vi "Cascade Controller.vi"(8 "error in":errorcluster) -> ()   [LabVIEW 2027]
doc: "This VI responds to drive commands both auto and tele Opmodes.\nIt owns the drivebase motors and sensors and runs independent from opModes. Commands can run for arbitrary times, but newly posted commands will interupt as long as Check is called and used for time delays."
uses:
  <vilib>/Rock Robotics/WPI/Framework/Completion Status.ctl
  Cascade Setpoints.ctl
  Cascade Operations.ctl
  Cascade Positions.ctl
  <vilib>/REV Custom Controls/SPARK Closed Loop Slot.ctl
  <vilib>/REV Custom Controls/Spark Output Control Type.ctl
  <vilib>/MRC/Types/CmdCtl Completion.ctl
  <vilib>/REVLibDriver/REVLibDriver.lvlib
  <resource>/objmgr/REVSpark.rc
  bef5a86c-5ad3-3fec-b018-693a5248eb3f.vi
panel:
  in  "Closed Loop Slot":T1 items=["Slot 0", "Slot 1", "Slot 2", "Slot 3"]
  in  "PID Gains":T2
  in  "PID Gains 2 VEL":T2={{"P Gain"=0.0001, "I Gain"=0.0, "D Gain"=0.0, "kV"=0.002}, "I Zone"=0.0, "Output LImits"={"Min Output"=-0.7, "Max Output"=0.7}}
  in  "PID Gains POS":T2
  in  "Abort Cmd":bool
  in  "Execute Cmd":bool
  in  "Interactive Values":T3
  out "Command Timing":cluster{"Start Time (ms)":u32, "Iterations":i32}
  out "Status":T6
  out "Current Command Data":T3
  out "Cmd Summary":string
  # "Interactive Command: You may fill in the settings for a command\nand schedule it with the Execute button. You can observe and abort\nany command while fine tuning the code for the controller."
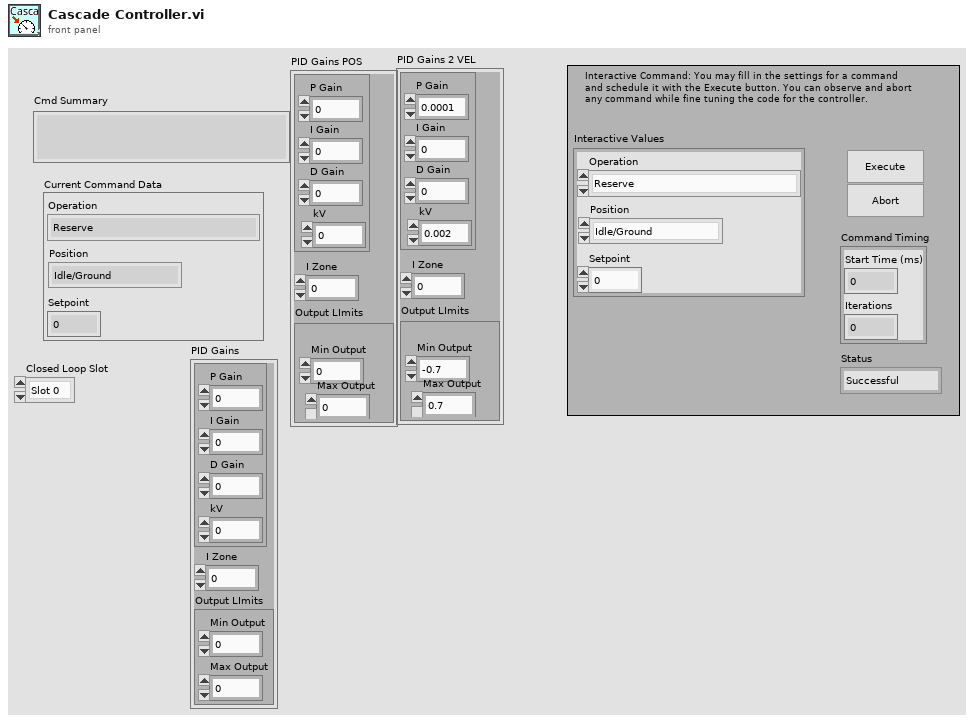
[diagram p1: front panel]
types:
  T1 = typedef "SPARK Closed Loop Slot.ctl" = u16
  T2 = cluster{cluster{"P Gain":dbl, "I Gain":dbl, "D Gain":dbl, "kV":dbl}, "I Zone":dbl, "Output LImits":cluster{"Min Output":dbl, "Max Output":dbl}}
  T3 = typedef "Cascade Setpoints.ctl" = cluster{"Operation":T4, "Position":T5, "Setpoint":dbl}
  T4 = typedef "Cascade Operations.ctl" = enum16{"Reserve", "Read Current", "Immediate", "State Machine"}
  T5 = typedef "Cascade Positions.ctl" = enum16{"Idle/Ground", "Raised L1", "L2", "L2 Tip", "L3", "L3 Tip", "Feeder", "\"Default\""}
  T6 = typedef "Completion Status.ctl" = enum16{"Successful", "Aborted", "Incomplete"}
  T7 = typedef "REVLibDriver.lvlib/REVSparkRefnum.ctl" = refnum<k20>
  T8 = typedef "Command Status Info.ctl" = cluster{"Name":string, "Status":T6, "notifier out":T9}
  T9 = typedef "Completion Notifier.ctl" = refnum<notifier>
  T10 = cluster{"Current Command":T3, "Command Timing":cluster{"Start Time (ms)":u32, "Iterations":i32}, "Command Arguments":cluster{"Command Info":T8, "Description":string, "Default Command":T3, "queue out":refnum<queue>, "Subsystem Name":string}}
  T11 = typedef "REVLibDriver.lvlib/Spark Output Control Type.ctl" = enum16{"Percent VBus", "Velocity", "Voltage", "Position", "Current", "MAXMotion Position", "MAXMotion Velocity"}
  T12 = typedef "CmdCtl Completion.ctl" = enum16{"incomplete", "finished"}
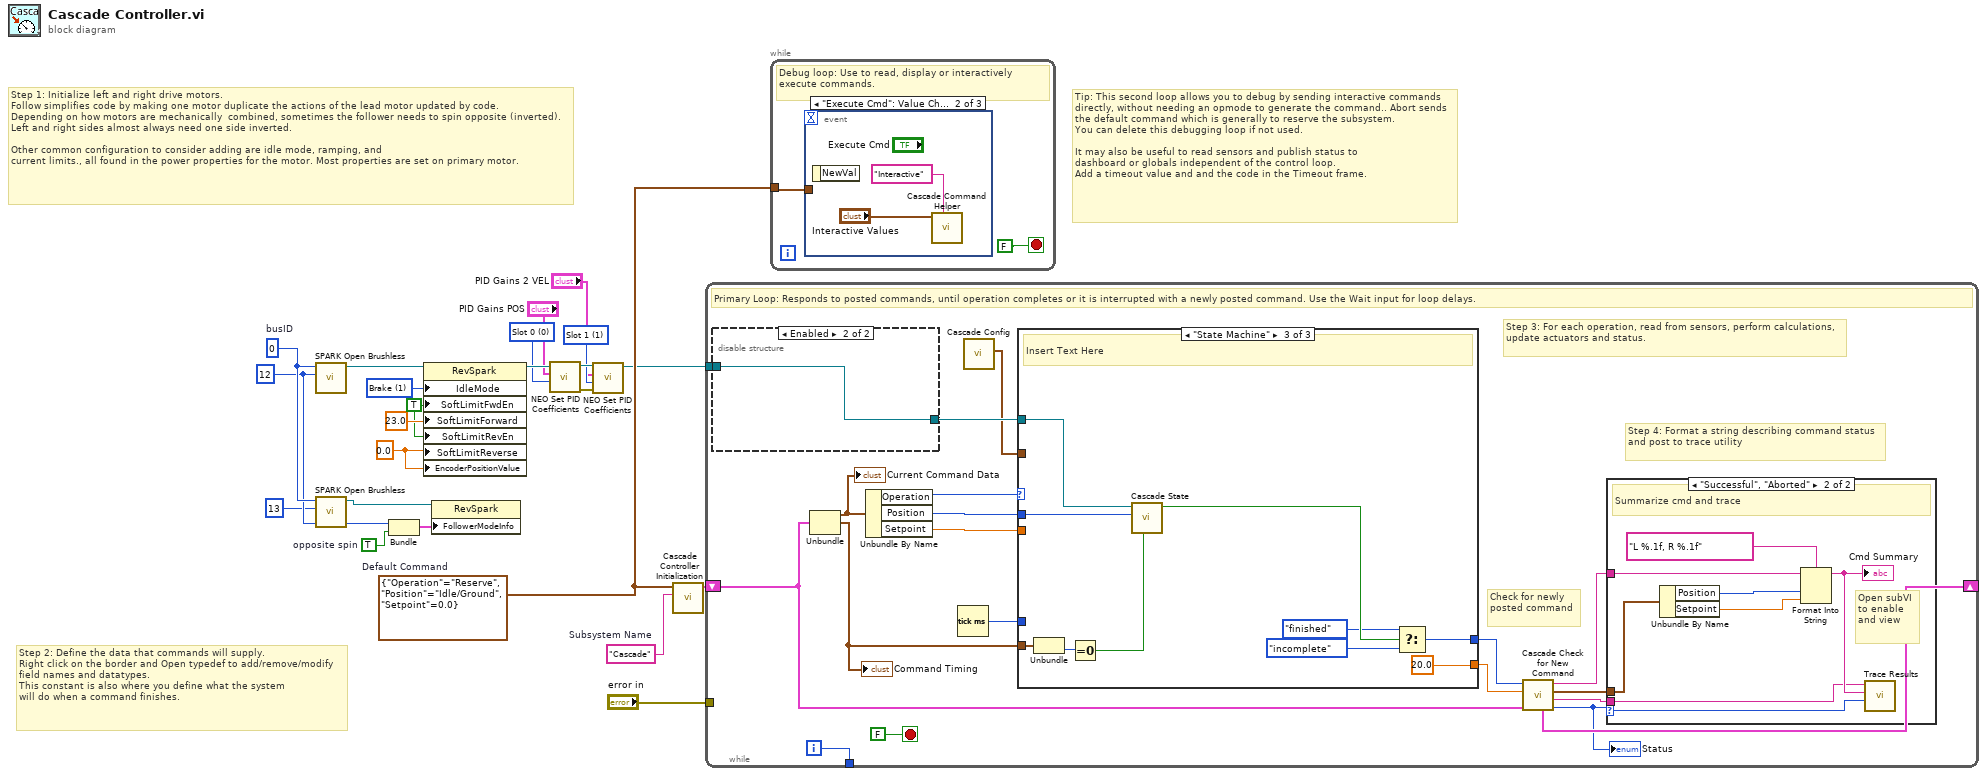
[diagram p0: block diagram]
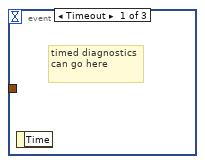
[diagram p2: hidden frame]
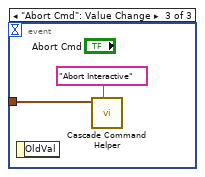
[diagram p3: hidden frame]
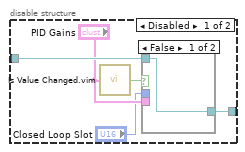
[diagram p4: hidden frame]
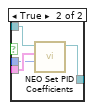
[diagram p5: hidden frame]
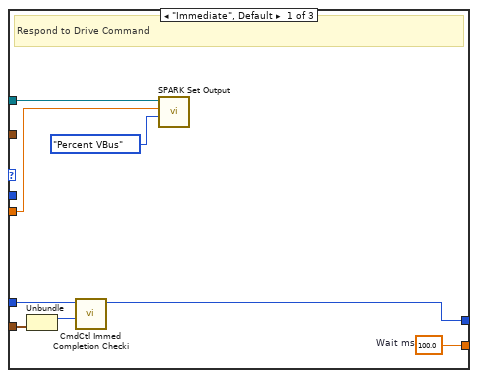
[diagram p7: hidden frame]
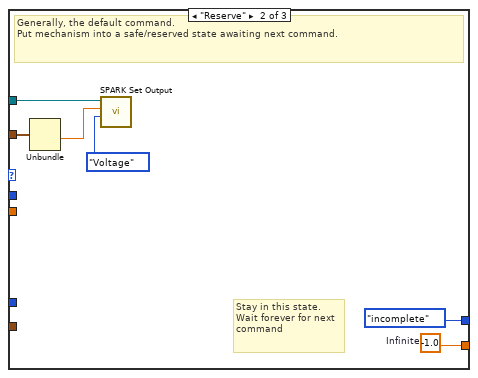
[diagram p8: hidden frame]
diagram:
  w5 = T1 1 items=["Slot 0", "Slot 1", "Slot 2", "Slot 3"] ("Closed Loop Slot")
  w2 = sgl 0.0 ("SoftLimitReverse")
  w1 = TRUE ("SoftLimitFwdEn")
  w10 = T1 0 items=["Slot 0", "Slot 1", "Slot 2", "Slot 3"] ("Closed Loop Slot")
  w12 = u32 1 items=["Coast", "Brake"] ("IdleMode")
  w17 = TRUE  # opposite spin
  w20 = 0  # busID
  w14 = 12
  w19 = T3 {"Operation"=enum."Reserve", "Position"=enum."Idle/Ground", "Setpoint"=0.0}  # Default Command
  w21 = "Cascade"  # Subsystem Name
  # "Tip: This second loop allows you to debug by sending interactive commands\ndirectly, without needing an opmode to generate the command.. Abort sends\nthe default command which is generally to reserve the subsystem.\nYou can delete this debugging loop if not used.\n\nIt may also be useful to read sensors and publish status to\ndashboard or globals independent of the control loop.\nAdd a timeout value and and the code in the Timeout frame."
  # "Step 2: Define the data that commands will supply.\nRight click on the border and Open typedef to add/remove/modify\nfield names and datatypes.\nThis constant is also where you define what the system\nwill do when a command finishes."
  # "Step 1: Initialize left and right drive motors.\nFollow simplifies code by making one motor duplicate the actions of the lead motor updated by code.\nDepending on how motors are mechanically  combined, sometimes the follower needs to spin opposite (inverted).\nLeft and right sides almost always need one side inverted.\n\nOther common configuration to consider adding are idle mode, ramping, and\ncurrent limits., all found in the power properties for the motor. Most properties are set on primary motor."
  n1 = call <vilib>:"SPARK Open Brushless.vi"("deviceId"=w14, "busID"=w20) -> ("Spark refnum"=w18:T7)  [unwired: 8 in, 1 out]
  n2 = call <vilib>:"SPARK Open Brushless.vi"("deviceId"=13, "busID"=w20) -> ("Spark refnum"=w16:T7)  [unwired: 8 in, 1 out]
  n3 = Bundle(w14, "opposite spin"=w17) -> (w15:cluster{i32, "opposite spin ":bool})  [unwired: 1 in]
  n4 = property class="RevSpark"(reference=w18, "IdleMode"=w12, "SoftLimitFwdEn"=w1, "SoftLimitForward"=sgl 23.0, "SoftLimitRevEn"=w1, "SoftLimitReverse"=w2, "EncoderPositionValue"=w2) -> (reference out=w11:T7)  [unwired: 1 in, 1 out]
  n5 = property class="RevSpark"(reference=w16, "FollowerModeInfo"=w15) -> ()  [unwired: 1 in, 2 out]
  n6 = call "NEO Set PID Coefficients.vi"("Closed Loop Slot"=w10, "PID Gains"="PID Gains POS", "Spark refnum"=w11) -> ("error out"=w7:errorcluster, "Spark refnum out"=w6:T7)  [unwired: 5 in]
  n7 = call "NEO Set PID Coefficients.vi"("error in"=w7, "Closed Loop Slot"=w5, "PID Gains"="PID Gains 2 VEL", "Spark refnum"=w6) -> ("Spark refnum out"=w3:T7)  [unwired: 4 in, 1 out]
  n8 = call "Cascade Controller Initialization.vi"("Subsystem Name"=w21, "Default Command"=w19) -> ("Current Command"=w22:T10)  [unwired: 9 in]
  n9 = while {
    shift-right: [w36] -> _
    shift-left: w22 -> [w30]
    tunnel: [w41] -> _
    tunnel: "error in" -> [_]
    tunnel: w3 -> [w26]
    i -> [w41]
    stop <- FALSE stop-if-true
    # "Step 4: Format a string describing command status\nand post to trace utility"
    # "Check for newly\nposted command"
    # "Step 3: For each operation, read from sensors, perform calculations,\nupdate actuators and status."
    # "Primary Loop: Responds to posted commands, until operation completes or it is interrupted with a newly posted command. Use the Wait input for loop delays."
    n10 = disable-structure shown="Enabled" {
      disable-tunnel: w26 -> [w47 w53]
      disable-tunnel: [w46 w53] -> w25
      frame Disabled {
        n11 = call "Is Value Changed.vim"("value"="PID Gains") -> ("changed or first call?"=w45:bool)
        n12 = case shown="False" w45 {
          tunnel: w47 -> [w48 w52]
          tunnel: [w48 w51] -> w46
          tunnel: "PID Gains" -> [_ w50]
          tunnel: "Closed Loop Slot" -> [_ w49]
          frame False {
          }
          frame True {
            n13 = call "NEO Set PID Coefficients.vi"("Closed Loop Slot"=w49, "PID Gains"=w50, "Spark refnum"=w52) -> ("Spark refnum out"=w51:T7)  [unwired: 5 in, 1 out]
          }
        }
      }
      frame Enabled {
      }
    }
    n14 = Unbundle(w30) -> ("Current Command"=w28:T3, "Command Timing"=w29:cluster{"Start Time (ms)":u32, "Iterations":i32})  [unwired: 1 out]
    "Command Timing" <- w29
    "Current Command Data" <- w28
    n15 = Unbundle By Name(w28) -> ("Operation"=w40:T4, "Position"=w39:T5, "Setpoint"=w37:dbl)
    n16 = Tick Count (ms)() -> (millisecond timer value=w38:u32)
    n17 = call "Cascade Config.vi"() -> ("FeedForward Constants Out"=w24:cluster{"kA":dbl, "kS":dbl, "kG":dbl, "kV":dbl})  [unwired: 10 in, 1 out]
    n18 = case shown="\"State Machine\"" w40 {
      tunnel: [w69 w75 20.0 ("Infinite")] -> w34
      tunnel: [w66 CmdCtl_Completion."incomplete" w81] -> w35
      tunnel: w29 -> [w68 _ w78]
      tunnel: w39 -> [_ _ w79]
      tunnel: w38 -> [w67 _ _]
      tunnel: w37 -> [w62 _ _]
      tunnel: w25 -> [w63 w73 w85]
      tunnel: w24 -> [_ w72 _]
      frame "Immediate", Default {
        w69 = 100.0  # Wait ms
        # "Respond to Drive Command"
        n19 = Unbundle(w68) -> ("Start Time (ms)"=w65:u32)  [unwired: 1 out]
        n20 = call <vilib>:"CmdCtl Immed Completion Checki.vi"("Start Time (ms)"=w65, "current time (ms)"=w67) -> ("Completion"=w66:T12)  [unwired: 9 in]
        n21 = call <vilib>:"SPARK Set Output.vi"("Control Mode"=Spark_Output_Control_Type."Percent VBus", "Setpoint"=w62, "Spark refnum"=w63) -> ()  [unwired: 7 in, 2 out]
      }
      frame "Reserve" {
        w75 = -1.0  # Infinite
        # "Stay in this state.\nWait forever for next\ncommand"
        # "Generally, the default command.\nPut mechanism into a safe/reserved state awaiting next command."
        n22 = Unbundle(w72) -> ("kG"=w71:dbl)  [unwired: 3 out]
        n23 = call <vilib>:"SPARK Set Output.vi"("Control Mode"=Spark_Output_Control_Type."Voltage", "Setpoint"=w71, "Spark refnum"=w73) -> ()  [unwired: 7 in, 2 out]
      }
      frame "State Machine" {
        # "Insert Text Here"
        n24 = Unbundle(w78) -> ("Iterations"=w77:i32)  [unwired: 1 out]
        n25 = Equal To 0?(x=w77) -> (x = 0?=w76:bool)
        n26 = call "Cascade State.vi"("First Iteration?"=w76, "Positions"=w79, "Cascade Motors"=w85) -> ("Is Finished?"=w84:bool)  [unwired: 8 in]
        n27 = Select(t=CmdCtl_Completion."finished", s=w84, f=CmdCtl_Completion."incomplete") -> (s? t:f=w81:T12)
      }
    }
    n28 = call "Cascade Check for New Command.vi"("Current Command"=w30, "Wait time (ms)"=w34, "Completion"=w35) -> ("Completion"=w27:T6, "Subsystem Name"=w31:string, "Current Command"=w32:T3, "Initial Trace String"=w33:string, "NextCommand"=w36:T10)  [unwired: 4 in]
    "Status" <- w27
    n29 = case shown="\"Successful\", \"Aborted\"" w27 {
      selector: w27 -> [_ w61]
      tunnel: w33 -> [_ w57]
      tunnel: w32 -> [_ w58]
      tunnel: w31 -> [_ w54]
      frame "Incomplete", Default {
        # "Continuing current command"
      }
      frame "Successful", "Aborted" {
        # "Open subVI\nto enable\nand view"
        # "Summarize cmd and trace"
        n30 = Unbundle By Name(w58) -> ("Position"=w60:T5, "Setpoint"=w55:dbl)
        n31 = Format Into String(format string="L %.1f, R %.1f", initial string=w57, w60, w55) -> (resulting string=w56:string)  [unwired: 1 in, 1 out]
        "Cmd Summary" <- w56
        n32 = call <vilib>:"Trace Results.vi"("Status of previous command"=w61, "Description"=w56, "Subsystem"=w54) -> ()  [unwired: 9 in]
      }
    }
  }
  n33 = while {
    tunnel: w19 -> [w86]
    stop <- FALSE stop-if-true
    # "Debug loop: Use to read, display or interactively execute commands."
    n34 = event shown="[1] \"Execute Cmd\": Value Change" {
      selector: _ -> [_ _ _]
      dyn-events: _ -> [_ _ _]
      timeout: _ -> [_ _ _]
      tunnel: w86 -> [_ _ w91]
      event Timeout {
        # "timed diagnostics\ncan go here"
        # "Insert Text Here"
        n35 = event-data() -> ()  [unwired: 1 in, 1 out]
      }
      event "Execute Cmd": Value Change {
        # "Execute"
        n36 = event-data() -> ()  [unwired: 1 in, 1 out]
        n37 = call "Cascade Command Helper.vi"("Description"="Interactive", "SubSystem Data"="Interactive Values") -> ()  [unwired: 7 in, 3 out]
      }
      event "Abort Cmd": Value Change {
        # "Insert Text Here"
        n38 = event-data() -> ()  [unwired: 1 in, 1 out]
        n39 = call "Cascade Command Helper.vi"("Description"="Abort Interactive", "SubSystem Data"=w91) -> ()  [unwired: 7 in, 3 out]
      }
    }
  }
